vi "Transport.showUI.vi"(8 "error in (no error)":errorcluster, 9 "Action":enum16{"Open", "Close"}(ring), 10 "method":T1=enum."LockinTimeDelay", 11 "Transport":refnum<class "Transport.lvclass">) -> (0 "error out":errorcluster)   [LabVIEW 2019, in "Transport.lvclass"]
uses:
  Transport.lvclass
  Typedefs/Transport.Methods--Enum.ctl
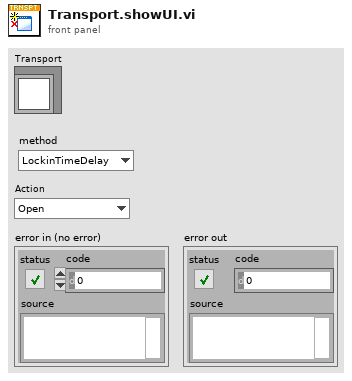
[diagram p1: front panel]
types:
  T1 = typedef "Transport.lvclass/Transport.Methods--Enum.ctl" = enum16{"LockinSweep", "LockinTime", "LockinTimeDelay"}
  T2 = enum32{"Invalid", "Standard", "Closed", "Hidden", "Minimized", "Maximized"}
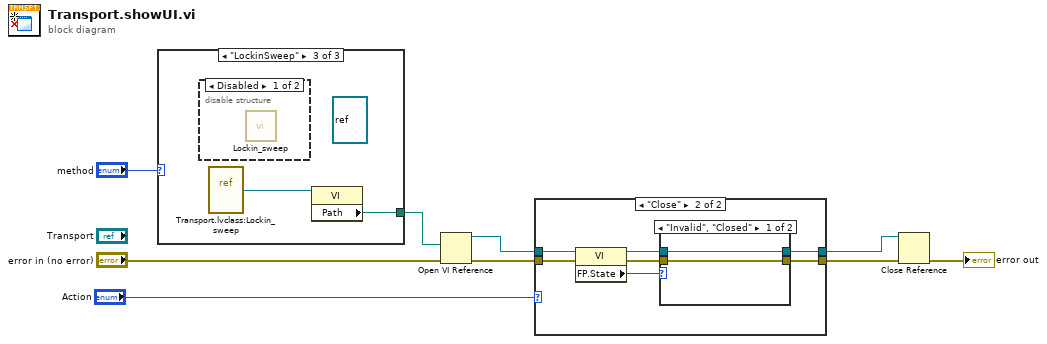
[diagram p0: block diagram]
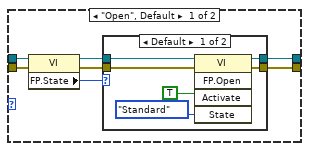
[diagram p2: hidden frame]
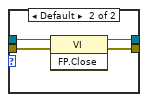
[diagram p4: hidden frame]
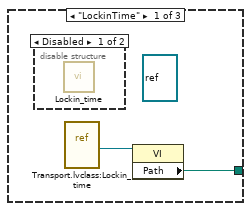
[diagram p5: hidden frame]
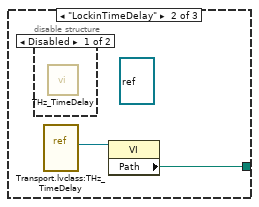
[diagram p7: hidden frame]
diagram:
  n1 = case shown="\"LockinSweep\"" "method" {
    tunnel: [w10 w12 w14] -> w8
    frame "LockinTime" {
      (unwired) refnum<vi> refnum ("type specifier VI Refnum (for type only)")
      n2 = disable-structure shown="Disabled" {
        frame Disabled {
          n3 = call "Lockin_time.vi"() -> ()  [unwired: 10 in, 2 out]
        }
        frame Enabled {
        }
      }
      n4 = vi-ref "Transport.lvclass:Lockin_time.vi"() -> (w11:refnum<vi>)
      n5 = property class="VI"(reference=w11) -> ("Path"=w10:path)  [unwired: 1 in, 2 out]
    }
    frame "LockinTimeDelay" {
      (unwired) refnum<vi> refnum ("type specifier VI Refnum (for type only)")
      n6 = disable-structure shown="Disabled" {
        frame Disabled {
          n7 = call "THz_TimeDelay.vi"() -> ()  [unwired: 10 in, 2 out]
        }
        frame Enabled {
        }
      }
      n8 = vi-ref "Transport.lvclass:THz_TimeDelay.vi"() -> (w13:refnum<vi>)
      n9 = property class="VI"(reference=w13) -> ("Path"=w12:path)  [unwired: 1 in, 2 out]
    }
    frame "LockinSweep" {
      (unwired) refnum<vi> refnum ("type specifier VI Refnum (for type only)")
      n10 = disable-structure shown="Disabled" {
        frame Disabled {
          n11 = call "Lockin_sweep.vi"() -> ()  [unwired: 9 in, 2 out]
        }
        frame Enabled {
        }
      }
      n12 = vi-ref "Transport.lvclass:Lockin_sweep.vi"() -> (w15:refnum<vi>)
      n13 = property class="VI"(reference=w15) -> ("Path"=w14:path)  [unwired: 1 in, 2 out]
    }
  }
  n14 = Open VI Reference(vi path=w8, error in (no error)="error in (no error)") -> (vi reference=w6:refnum<vi>, error out=w7:errorcluster)  [unwired: 4 in]
  n15 = case shown="\"Close\"" "Action" {
    tunnel: w7 -> [w20 w36]
    tunnel: [w22 w37] -> w3
    tunnel: w6 -> [w21 w34]
    tunnel: [w16 w31] -> w5
    frame "Open", Default {
      n16 = property class="VI"(reference=w21, error in=w20) -> (reference out=w18:refnum<vi>, error out=w19:errorcluster, "FP.State"=w17:T2)
      n17 = case shown="Default" w17 {
        tunnel: [w26 w30] -> w22
        tunnel: w19 -> [w25 w30]
        tunnel: w18 -> [w24 w29]
        tunnel: [w23 w29] -> w16
        frame Default {
          n18 = invoke class="VI" method="FP.Open"(reference=w24, error in=w25, "Activate"=TRUE, "State"=T2."Standard") -> (reference out=w23:refnum<vi>, error out=w26:errorcluster)  [unwired: 1 in, 3 out]
        }
        frame "Invalid" {
        }
      }
    }
    frame "Close" {
      n19 = property class="VI"(reference=w34, error in=w36) -> (reference out=w33:refnum<vi>, error out=w35:errorcluster, "FP.State"=w32:T2)
      n20 = case shown="\"Invalid\", \"Closed\"" w32 {
        tunnel: [w39 w43] -> w37
        tunnel: w35 -> [w39 w42]
        tunnel: w33 -> [w38 w41]
        tunnel: [w38 w40] -> w31
        frame "Invalid", "Closed" {
        }
        frame Default {
          n21 = invoke class="VI" method="FP.Close"(reference=w41, error in=w42) -> (reference out=w40:refnum<vi>, error out=w43:errorcluster)  [unwired: 1 in, 1 out]
        }
      }
    }
  }
  n22 = Close Reference(reference=w5, error in (no error)=w3) -> (error out=→"error out":errorcluster)
